vi "Relative Path Default.vi"(0 "path input":path=path "WireLint/default.txt", 11 "error in":errorcluster) -> (4 "path text":string, 15 "error out":errorcluster)   [LabVIEW 2024]
doc: "Fixture containing one path control with a relative default."
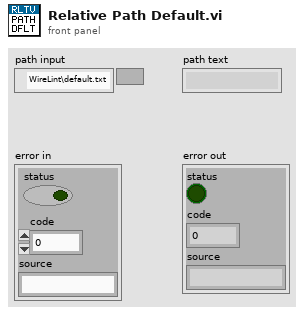
[diagram p1: front panel]
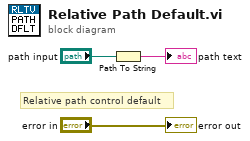
[diagram p0: block diagram]
diagram:
  # "Relative path control default"
  n1 = Path To String(path="path input") -> (string=→"path text":string)
  "error out" <- "error in"
